vi "MouseClick.vi"(11 "Error In":errorcluster, 13 "ClickFunction":T1) -> (15 "Error Out":errorcluster)   [LabVIEW 2019, in "Drona.lvlib"]
doc: "This VI simulates mouse right click action"
uses:
  Drona.lvlib
  Controls/ClickFunction.ctl
  user32.dll
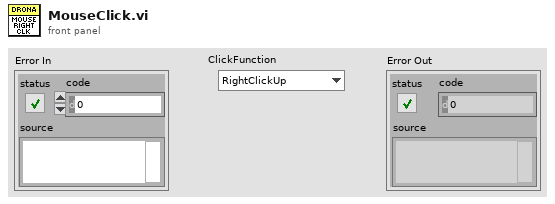
[diagram p1: front panel]
types:
  T1 = typedef "Drona.lvlib/ClickFunction.ctl" = enum16{"RightClickUp", "RightClickDown", "LeftClickUp", "LeftClickDown"}
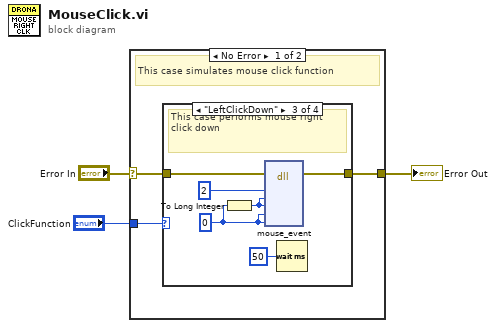
[diagram p0: block diagram]
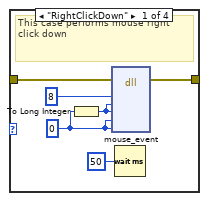
[diagram p2: hidden frame]
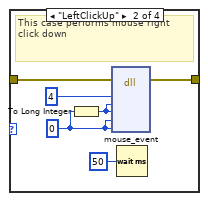
[diagram p3: hidden frame]
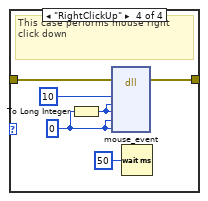
[diagram p4: hidden frame]
diagram:
  n1 = case shown="No Error" "Error In" {
    selector: "Error In" -> [w6 w31]
    tunnel: [w5 w31] -> w1
    tunnel: "ClickFunction" -> [w4 _]
    frame No Error {
      # "This case simulates mouse click function"
      n2 = case shown="\"LeftClickDown\"" w4 {
        tunnel: w6 -> [w12 w18 w24 w30]
        tunnel: [w11 w17 w23 w29] -> w5
        frame "RightClickDown" {
          w9 = u32 0 ("dwExtraInfo")
          # "This case performs mouse right click down"
          n3 = To Long Integer(number=w9) -> (32bit integer=w8:i32)
          n4 = dll-call lib="user32.dll" fn="mouse_event"(error in=w12, "dwFlags"=8, "dx"=w8, "dy"=w8, "dwData"=w9, "dwExtraInfo"=w9) -> (error out=w11:errorcluster)  [unwired: 8 in, 1 out]
          n5 = Wait (ms)(milliseconds to wait=u32 50) -> ()  [unwired: 1 out]
        }
        frame "LeftClickUp" {
          w15 = u32 0 ("dwExtraInfo")
          # "This case performs mouse right click down"
          n6 = To Long Integer(number=w15) -> (32bit integer=w14:i32)
          n7 = dll-call lib="user32.dll" fn="mouse_event"(error in=w18, "dwFlags"=4, "dx"=w14, "dy"=w14, "dwData"=w15, "dwExtraInfo"=w15) -> (error out=w17:errorcluster)  [unwired: 8 in, 1 out]
          n8 = Wait (ms)(milliseconds to wait=u32 50) -> ()  [unwired: 1 out]
        }
        frame "LeftClickDown" {
          w21 = u32 0 ("dwExtraInfo")
          # "This case performs mouse right click down"
          n9 = To Long Integer(number=w21) -> (32bit integer=w20:i32)
          n10 = dll-call lib="user32.dll" fn="mouse_event"(error in=w24, "dwFlags"=2, "dx"=w20, "dy"=w20, "dwData"=w21, "dwExtraInfo"=w21) -> (error out=w23:errorcluster)  [unwired: 8 in, 1 out]
          n11 = Wait (ms)(milliseconds to wait=u32 50) -> ()  [unwired: 1 out]
        }
        frame "RightClickUp" {
          w27 = u32 0 ("dwExtraInfo")
          # "This case performs mouse right click down"
          n12 = To Long Integer(number=w27) -> (32bit integer=w26:i32)
          n13 = dll-call lib="user32.dll" fn="mouse_event"(error in=w30, "dwFlags"=10, "dx"=w26, "dy"=w26, "dwData"=w27, "dwExtraInfo"=w27) -> (error out=w29:errorcluster)  [unwired: 8 in, 1 out]
          n14 = Wait (ms)(milliseconds to wait=u32 50) -> ()  [unwired: 1 out]
        }
      }
    }
    frame Error {
      # "If error, this case pass that error message only"
    }
  }
  "Error Out" <- w1
